vi "Populate Single Example Description.vi"(6 "Show FP":bool, 8 "error in (no error)":errorcluster, 10 "VI Description":string, 11 "Path":path) -> (0 "error out":errorcluster)   [LabVIEW 2017, in "csmdoc.lvlib"]
uses:
  csmdoc.lvlib
  _Shared/CSM Shared.lvlib
  _tool/_file/csm-file-support.lvlib
  Communicable State Machine.lvlib
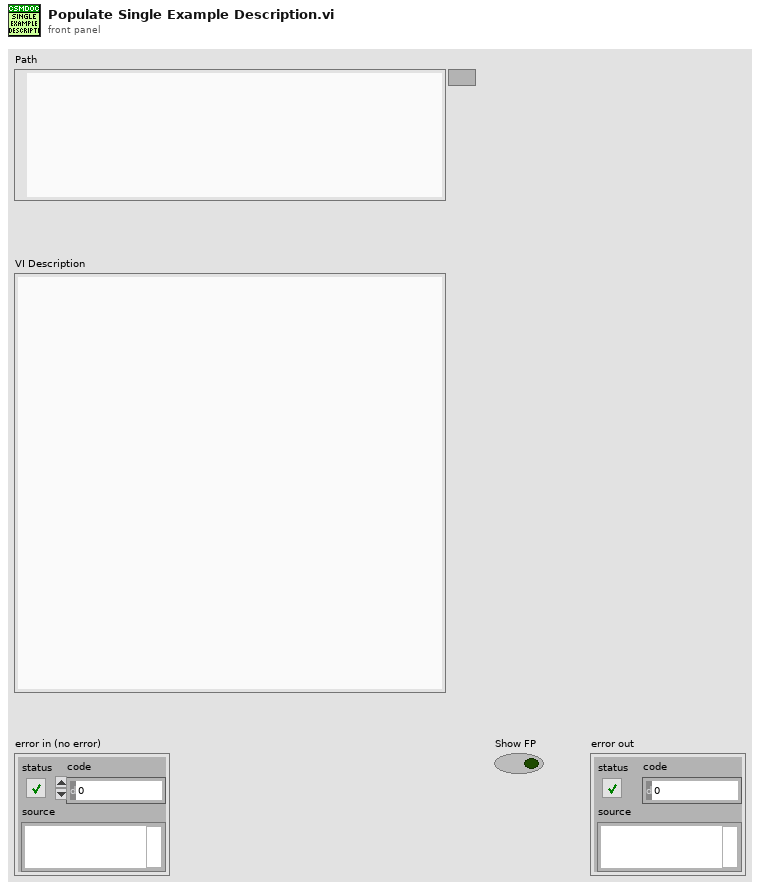
[diagram p1: front panel]
types:
  T1 = typedef "csmdoc.lvlib/DocElement.ctl" = cluster{"ID":string, "Content":string[], "SubIDs":string[], "Path":string[]}
  T2 = typedef "csmdoc.lvlib/DocNote.ctl" = cluster{"ID":string, "Content":string, "Type":string}
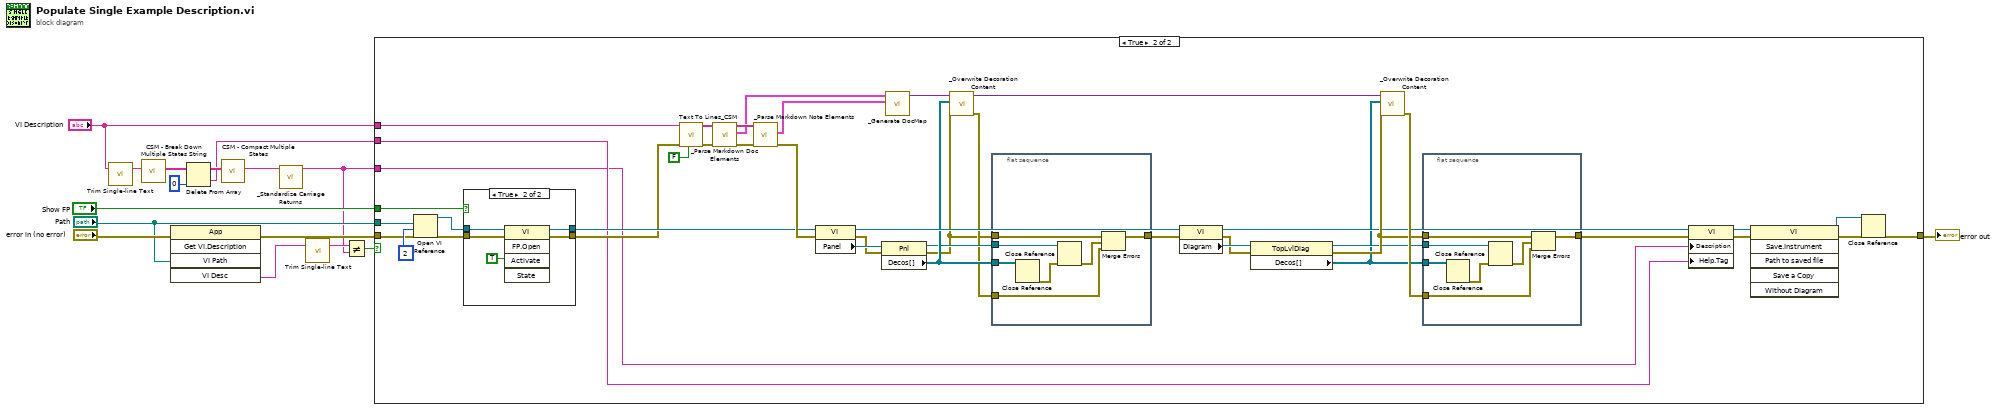
[diagram p0: block diagram]
diagram:
  n1 = call "Trim Single-line Text.vi"("single-line text"="VI Description") -> ("trimed text"=w8:string)  [unwired: 2 in]
  n2 = call "CSM - Break Down Multiple States String.vi"("States"=w8) -> ("Multiple States"=w7:string[])  [unwired: 10 in]
  n3 = invoke class="App" method="Get VI.Description"(error in="error in (no error)", "VI Path"="Path") -> (error out=w16:errorcluster, "VI Desc"=w10:string)  [unwired: 3 in, 3 out]
  n4 = Delete From Array(array=w7, index=0) -> (deleted portion=w2:string, array with subset deleted=w5:string[])  [unwired: 1 in]
  n5 = call "CSM - Compact Multiple States.vi"("Multiple States"=w5) -> ("States"=w4:string)  [unwired: 9 in]
  n6 = call "_Standardize Carriage Returns.vi"("States"=w4) -> ("trimed text"=w1:string)  [unwired: 10 in]
  n7 = call "Trim Single-line Text.vi"("single-line text"=w10) -> ("trimed text"=w14:string)  [unwired: 2 in]
  n8 = Not Equal?(x=w14, y=w1) -> (x != y?=w15:bool)
  n9 = case shown="True" w15 {
    tunnel: w16 -> [w17 w55]
    tunnel: "VI Description" -> [_ w33]
    tunnel: [w17 w52] -> w12
    tunnel: "Show FP" -> [_ w59]
    tunnel: "Path" -> [_ w51]
    tunnel: w2 -> [_ w19]
    tunnel: w1 -> [_ w18]
    frame False {
    }
    frame True {
      n10 = Open VI Reference(vi path=w51, options=2, error in (no error)=w55) -> (vi reference=w56:refnum<vi>, error out=w57:errorcluster)  [unwired: 3 in]
      n11 = case shown="True" w59 {
        tunnel: w57 -> [w74 w79]
        tunnel: w56 -> [w75 w78]
        tunnel: [w74 w77] -> w34
        tunnel: [w75 w76] -> w35
        frame False {
        }
        frame True {
          n12 = invoke class="VI" method="FP.Open"(reference=w78, error in=w79, "Activate"=TRUE ("Activate?")) -> (reference out=w76:refnum<vi>, error out=w77:errorcluster)  [unwired: 2 in, 3 out]
        }
      }
      n13 = call "Text To Lines_CSM.vi"("Remove Empty Lines? (T)"=FALSE ("Remove Empty Lines?(T)"), "error in (no error)"=w34, "String"=w33) -> ("error out"=w48:errorcluster, "Lines"=w49:string[])  [unwired: 7 in]
      n14 = call "_Parse Markdown Doc Elements.vi"("Error in"=w48, "Lines"=w49) -> ("Error out"=w44:errorcluster, "Array"=w42:T1[], "Lines (dup)"=w45:string[])  [unwired: 7 in]
      n15 = call "_Parse Markdown Note Elements.vi"("Error in"=w44, "Lines"=w45) -> ("Error out"=w43:errorcluster, "Array"=w41:T2[])  [unwired: 7 in, 1 out]
      n16 = property class="VI"(reference=w35, error in=w43) -> (reference out=w46:refnum<vi>, error out=w37:errorcluster, "Panel"=w47:refnum<vi>)
      n17 = property class="Pnl"(reference=w47, error in=w37) -> (reference out=w39:refnum<vi>, error out=w31:errorcluster, "Decos[]"=w40:refnum<vi>[])
      n18 = call "_Generate DocMap.vi"("Array 2"=w41, "Array"=w42) -> ("Variant"=w36:variant)  [unwired: 9 in]
      n19 = call "_Overwrite Decoration Content.vi"("error in (no error)"=w31, "Decos[]"=w40, "Variant in"=w36) -> ("error out"=w32:errorcluster, "Variant out"=w25:variant)  [unwired: 7 in]
      n20 = flat-sequence {
        tunnel: w40 -> [w73]
        tunnel: w39 -> [w72]
        tunnel: [w70] -> w38
        tunnel: w31 -> [w68]
        tunnel: w32 -> [w67]
        frame #0 {
          n21 = Close Reference(reference=w73) -> (error out=w71:errorcluster)  [unwired: 1 in]
          n22 = Close Reference(reference=w72, error in (no error)=w71) -> (error out=w69:errorcluster)
          n23 = Merge Errors(w68, w69, w67) -> (w70:errorcluster)
        }
      }
      n24 = property class="VI"(reference=w46, error in=w38) -> (reference out=w24:refnum<vi>, error out=w29:errorcluster, "Diagram"=w30:refnum<vi>)
      n25 = property class="TopLvlDiag"(reference=w30, error in=w29) -> (reference out=w26:refnum<vi>, error out=w27:errorcluster, "Decos[]"=w22:refnum<vi>[])
      n26 = call "_Overwrite Decoration Content.vi"("error in (no error)"=w27, "Decos[]"=w22, "Variant in"=w25) -> ("error out"=w28:errorcluster)  [unwired: 7 in, 1 out]
      n27 = flat-sequence {
        tunnel: w22 -> [w66]
        tunnel: w26 -> [w65]
        tunnel: [w63] -> w23
        tunnel: w27 -> [w61]
        tunnel: w28 -> [w60]
        frame #0 {
          n28 = Close Reference(reference=w66) -> (error out=w64:errorcluster)  [unwired: 1 in]
          n29 = Close Reference(reference=w65, error in (no error)=w64) -> (error out=w62:errorcluster)
          n30 = Merge Errors(w61, w62, w60) -> (w63:errorcluster)
        }
      }
      n31 = property class="VI"(reference=w24, error in=w23, "Description"=w18, "Help.Tag"=w19) -> (reference out=w20:refnum<vi>, error out=w21:errorcluster)
      n32 = invoke class="VI" method="Save.Instrument"(reference=w20, error in=w21) -> (reference out=w53:refnum<vi>, error out=w54:errorcluster)  [unwired: 4 in, 4 out]
      n33 = Close Reference(reference=w53, error in (no error)=w54) -> (error out=w52:errorcluster)
    }
  }
  "error out" <- w12
